vi "create run for specific asset.vi"(9 "Start Time (now)":timestamp format="%<%x %.3X>T", 10 "Title":string, 11 "asset":refnum<class "asset.lvclass">) -> (0 "error out":errorcluster, 3 "Run":refnum<class "Run.lvclass">)   [LabVIEW 2020, in "nominal core steps.lvlib"]
doc: "Creates a run associated with a specific asset. Runs represent a time range and are required to have a start time."
uses:
  nominal core steps.lvlib
  <vilib>/Nominal/Nominal IO Client/lv_src/Run/Run.lvclass
  <vilib>/Nominal/Nominal IO Client/lv_src/asset/asset.lvclass
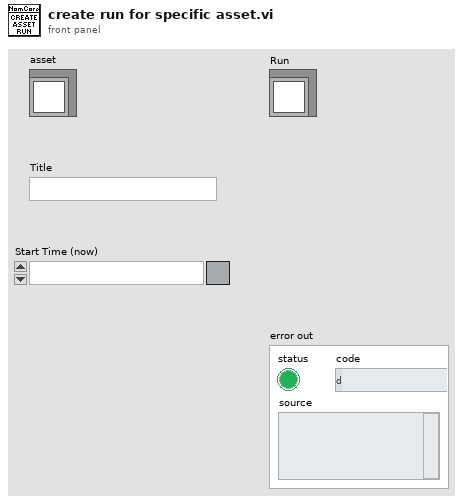
[diagram p1: front panel]
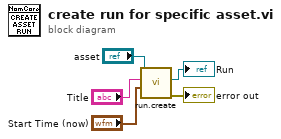
[diagram p0: block diagram]
diagram:
  n1 = call <vilib>:"run.create.vi"("Start Time (now)"="Start Time (now)", "Title"="Title", "asset in"="asset") -> ("error out"=→"error out":errorcluster, "Run"=→"Run":refnum<class "Run.lvclass">)  [unwired: 6 in, 1 out]
